vi "DumpSendEvent.vi"(6 "Data":dbl[][](array[numeric]), 9 "DumpFileAction":T1, 10 "Path":path, 11 "DumpFileQueue":T2) -> ()   [LabVIEW 2025]
uses:
  DumpFileQueue.ctl
  DumpFileEvent.ctl
  DumpFileAction.ctl
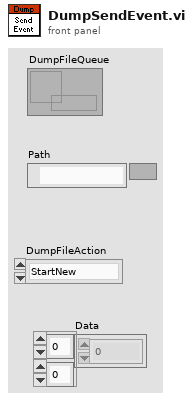
[diagram p1: front panel]
types:
  T1 = typedef "DumpFileAction.ctl" = enum16{"StartNew", "StartAppend", "Data", "Close"}
  T2 = typedef "DumpFileQueue.ctl" = refnum<queue>
  T3 = typedef "DumpFileEvent.ctl" = cluster{"Path":path, "DumpFileAction":T1, "Data":dbl[][]}
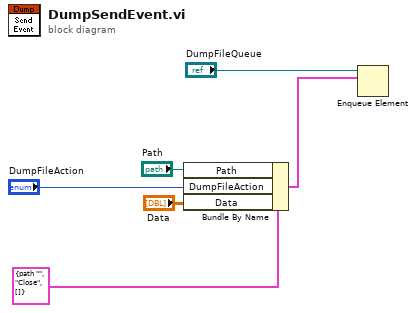
[diagram p0: block diagram]
diagram:
  n1 = Bundle By Name(cluster=T3 {"Path"=path "", "DumpFileAction"=enum."Close", "Data"=[]} ("element"), "Path"="Path", "DumpFileAction"="DumpFileAction", "Data"="Data") -> (w4:T3)
  n2 = Enqueue Element(queue="DumpFileQueue", element=w4) -> ()  [unwired: 2 in, 3 out]
